vi "Saturating Accumulator.vi"() -> ()   [LabVIEW 2026]
doc: "While-loop accumulator: each iteration adds Increment to a running total, saturating the total at Limit; counts iterations, flags whether saturation ever occurred, and records the per-iteration history as an array. The loop stops once the iteration count reaches Max Iterations. Self-contained: primitives, loops, case and shift registers only."
panel:
  out "History":dbl[](array[numeric])
  out "Saturated":bool
  out "Iterations":i32
  out "Final Value":dbl
  in  "Max Iterations":i32=8
  in  "Limit":dbl=10.0
  in  "Increment":dbl=1.5
  in  "Start Value":dbl
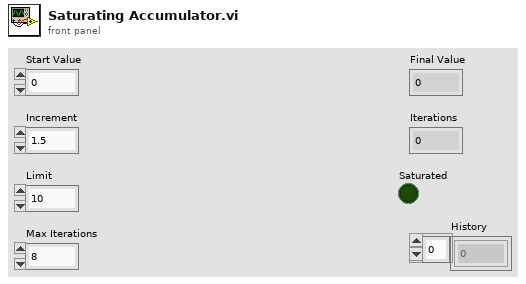
[diagram p1: front panel]
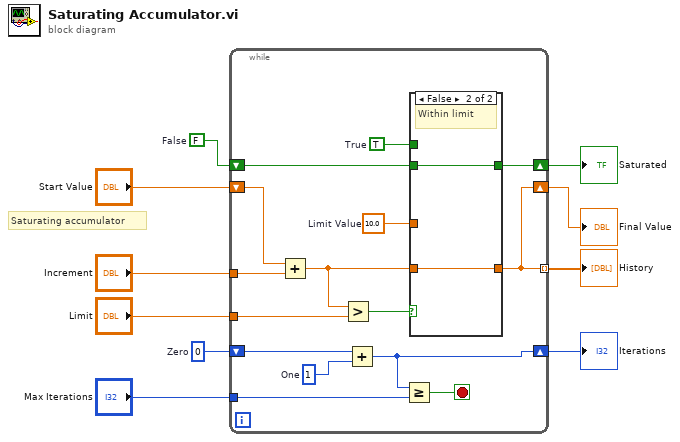
[diagram p0: block diagram]
diagram:
  w5 = FALSE  # False
  w6 = 0  # Zero
  # "Saturating accumulator"
  n1 = while {
    tunnel: "Increment" -> [w24]
    tunnel: "Limit" -> [w23]
    tunnel: "Max Iterations" -> [w19]
    shift-right: [w11] -> w4
    shift-left: "Start Value" -> [w25]
    shift-right: [w20] -> w3
    shift-left: w6 -> [w22]
    shift-right: [w13] -> w2
    shift-left: w5 -> [w14]
    tunnel: [w11] -> w1 mode=indexing
    stop <- w18 stop-if-true
    w21 = 1  # One
    w17 = 10.0  # Limit Value
    w16 = TRUE  # True
    n2 = Add(x=w25, y=w24) -> (x+y=w15:dbl)
    n3 = Greater?(x=w15, y=w23) -> (0:w12:bool)
    n4 = Add(x=w22, y=w21) -> (x+y=w20:i32)
    n5 = Greater Or Equal?(x=w20, y=w19) -> (x >= y?=w18:bool)
    n6 = case shown="False" w12 {
      tunnel: [w27 w29] -> w11
      tunnel: w17 -> [w27 _]
      tunnel: [w26 w28] -> w13
      tunnel: w16 -> [w26 _]
      tunnel: w15 -> [_ w29]
      tunnel: w14 -> [_ w28]
      frame True {
        # "Over limit"
      }
      frame False {
        # "Within limit"
      }
    }
  }
  "Final Value" <- w4
  "Iterations" <- w3
  "Saturated" <- w2
  "History" <- w1
